vi "Create and Register Sessions.vi"(8 "error in (no error)":errorcluster, 11 "Pinmap Path":string) -> (0 "error out":errorcluster)   [LabVIEW 2020, in "NIDCPowerSourceDCVoltage.lvlib"]
uses:
  NIDCPowerSourceDCVoltage.lvlib
  <vilib>/MeasurementLink/MeasurementLink Session Management Client/RPC Messages/ni_measurementlink_sessionmanagement_v1_ReserveSessionsRequest.ctl
  <vilib>/MeasurementLink/MeasurementLink Session Management Client/RPC Messages/ni_measurementlink_PinMapContext.ctl
  <vilib>/MeasurementLink/MeasurementLink Discovery Client/RPC Messages/ni_measurementlink_discovery_v1_ResolveServiceRequest.ctl
  <vilib>/MeasurementLink/MeasurementLink Session Management Client/MeasurementLink Session Management Client.lvlib
  <vilib>/MeasurementLink/MeasurementLink Discovery Client/MeasurementLink Discovery Client.lvlib
  <vilib>/MeasurementLink/MeasurementLink Measurement Server/MeasurementLink Measurement Server.lvlib
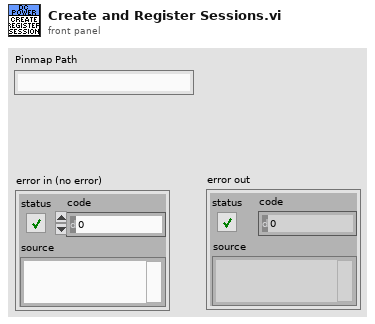
[diagram p1: front panel]
types:
  T1 = typedef "MeasurementLink Discovery Client.lvlib/ni_measurementlink_discovery_v1_ResolveServiceRequest.ctl" = cluster{"provided_interface":string, "service_class":string}
  T2 = typedef "MeasurementLink Session Management Client.lvlib/ni_measurementlink_sessionmanagement_v1_ReserveSessionsRequest.ctl" = cluster{"pin_map_context":T3, "pin_or_relay_names":string[], "instrument_type_id":string, "timeout_in_milliseconds":i32}
  T3 = typedef "MeasurementLink Session Management Client.lvlib/ni_measurementlink_PinMapContext.ctl" = cluster{"pin_map_id":string, "sites":i32[]}
  T4 = typedef "grpc-lvsupport-release.lvlib/grpcId.ctl" = u64
  T5 = typedef "MeasurementLink Discovery Client.lvlib/ni_measurementlink_discovery_v1_ServiceLocation.ctl" = cluster{"location":string, "insecure_port":string, "ssl_authenticated_port":string}
  T6 = typedef "MeasurementLink Session Management Client.lvlib/ni_measurementlink_sessionmanagement_v1_ReserveSessionsResponse.ctl" = cluster{"sessions":T7[]}
  T7 = typedef "MeasurementLink Session Management Client.lvlib/ni_measurementlink_sessionmanagement_v1_SessionInformation.ctl" = cluster{"session":T8, "resource_name":string, "channel_list":string, "instrument_type_id":string, "session_exists":bool, "channel_mappings":T9[]}
  T8 = typedef "MeasurementLink Session Management Client.lvlib/nidevice_grpc_Session.ctl" = cluster{"name":string}
  T9 = typedef "MeasurementLink Session Management Client.lvlib/ni_measurementlink_sessionmanagement_v1_ChannelMapping.ctl" = cluster{"pin_or_relay_name":string, "site":i32, "channel":string}
  T10 = typedef "niDCPower gRPC Device Server.ctl" = cluster{"session Name":string, "address (localhost)":string, "port (31763)":i32}
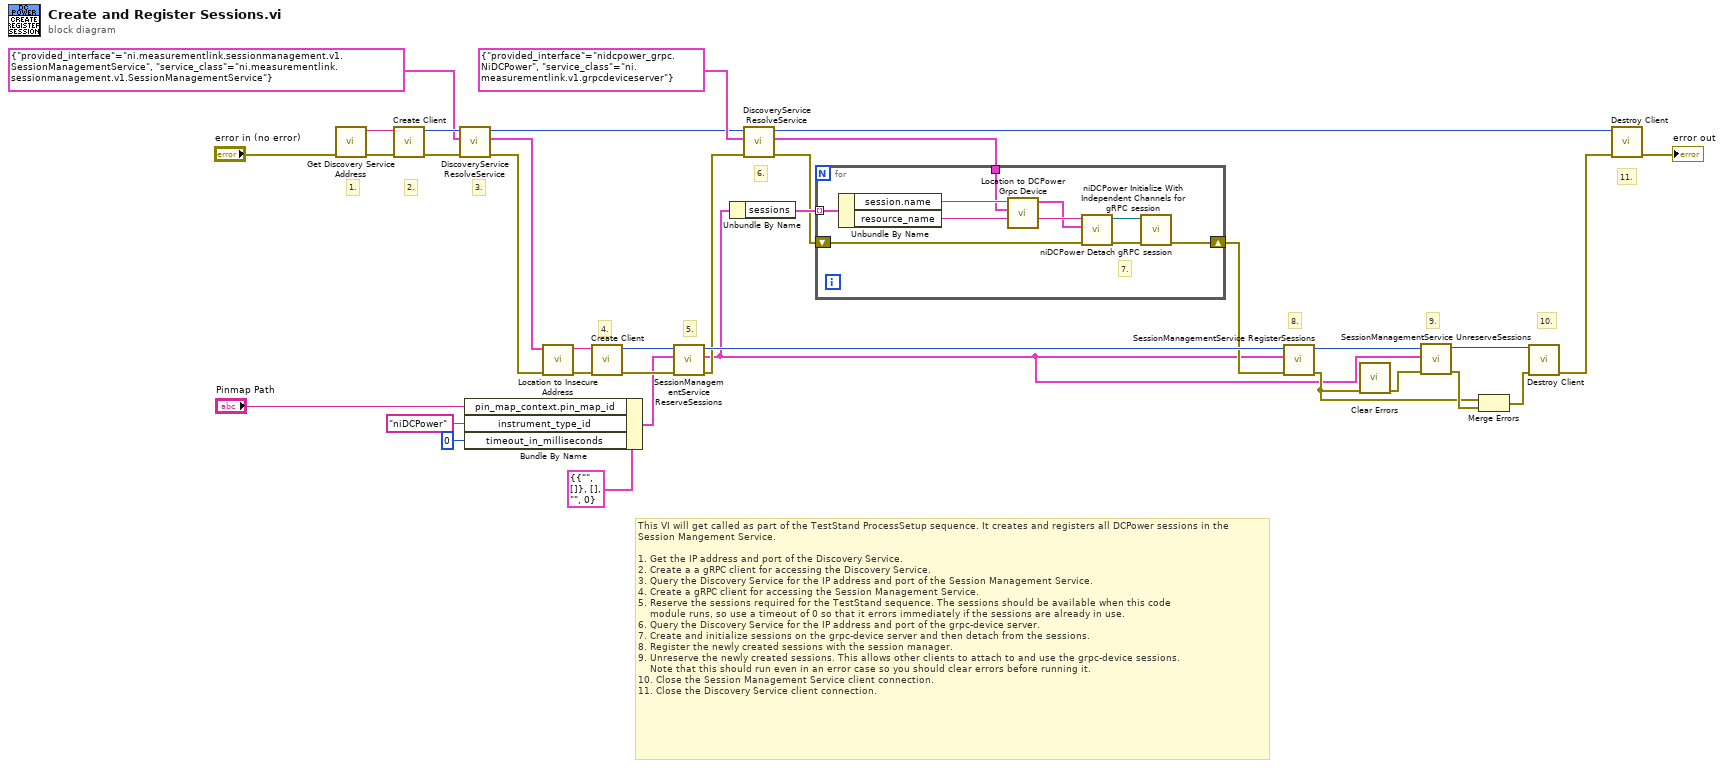
[diagram p0: block diagram]
diagram:
  # "11."
  # "10."
  # "9."
  # "8."
  # "6."
  # "5."
  # "4."
  # "3."
  # "2."
  # "1."
  # "This VI will get called as part of the TestStand ProcessSetup sequence. It creates and registers all DCPower sessions in the\nSession Mangement Service.\n\n1. Get the IP address and port of the Discovery Service.\n2. Create a a gRPC client for accessing the Discovery Service.\n3. Query the Discovery Service for the IP address and port of the Session Management Service.\n4. Create a gRPC client for accessing the Session Management Service.\n5. Reserve the sessions required for the TestStand sequence. The sessions should be available when this code\n    module runs, so use a timeout of 0 so that it errors immediately if the sessions are already in use.  \n6. Query the Discovery Service for the IP address and port of the grpc-device server.\n7. Create and initialize sessions on the grpc-device server and then detach from the sessions.\n8. Register the newly created sessions with the session manager.\n9. Unreserve the newly created sessions. This allows other clients to attach to and use the grpc-device sessions. \n    Note that this should run even in an error case so you should clear errors before running it.\n10. Close the Session Management Service client connection.\n11. Close the Discovery Service client connection."
  n1 = call <vilib>:"Get Discovery Service Address.vi"("error in"="error in (no error)") -> ("error out"=w10:errorcluster, "address"=w9:string)  [unwired: 9 in]
  n2 = call <vilib>:"Create Client.vi"("error in"=w10, "address"=w9) -> ("error out"=w30:errorcluster, "gRPC ID Out"=w31:T4)  [unwired: 8 in]
  n3 = call <vilib>:"DiscoveryService ResolveService.vi"("error in"=w30, "Request Data"=T1 {"provided_interface"="ni.measurementlink.sessionmanagement.v1.SessionManagementService", "service_class"="ni.measurementlink.sessionmanagement.v1.SessionManagementService"}, "gRPC ID"=w31) -> ("error out"=w29:errorcluster, "Response Data"=w8:T5, "gRPC ID out"=w17:T4)  [unwired: 6 in]
  n4 = Bundle By Name(cluster=T2 {"pin_map_context"={"pin_map_id"="", "sites"=[]}, "pin_or_relay_names"=[], "instrument_type_id"="", "timeout_in_milliseconds"=0} ("Request Data"), "pin_map_context.pin_map_id"="Pinmap Path", "instrument_type_id"="niDCPower", "timeout_in_milliseconds"=0) -> (w24:T2)
  n5 = call "Location to Insecure Address.vi"("Response Data"=w8) -> ("String"=w7:string)  [unwired: 10 in]
  n6 = call <vilib>:"Create Client.vi"("error in"=w29, "address"=w7) -> ("error out"=w33:errorcluster, "gRPC ID Out"=w34:T4)  [unwired: 8 in]
  n7 = call <vilib>:"SessionManagementService ReserveSessions.vi"("error in"=w33, "Request Data"=w24, "gRPC ID"=w34) -> ("error out"=w15:errorcluster, "Response Data"=w2:T6, "gRPC ID out"=w32:T4)  [unwired: 6 in]
  n8 = Unbundle By Name(w2) -> ("sessions"=w19:T7[])
  n9 = call <vilib>:"DiscoveryService ResolveService.vi"("error in"=w15, "Request Data"=T1 {"provided_interface"="nidcpower_grpc.NiDCPower", "service_class"="ni.measurementlink.v1.grpcdeviceserver"}, "gRPC ID"=w17) -> ("error out"=w14:errorcluster, "Response Data"=w13:T5, "gRPC ID out"=w16:T4)  [unwired: 6 in]
  n10 = for {
    tunnel: w19 -> [w40] mode=indexing
    shift-right: [w42] -> w22
    shift-left: w14 -> [w43]
    tunnel: w13 -> [w38]
    # "7."
    n11 = Unbundle By Name(w40) -> ("session.name"=w39:string, "resource_name"=w41:string)
    n12 = call "Location to DCPower Grpc Device.vi"("Grpc Device Location"=w38, "Session Name"=w39) -> ("NI gRPC Device Server Out"=w35:T10)  [unwired: 9 in]
    n13 = call <instrlib>:"niDCPower Initialize With Independent Channels for gRPC session.vi"("error in (no error)"=w43, "NI gRPC Device Server"=w35, "resource name"=w41) -> ("error out"=w37:errorcluster, "instrument handle out"=w36:refnum<k15>)  [unwired: 7 in]
    n14 = call <instrlib>:"niDCPower Detach gRPC session.vi"("error in (no error)"=w37, "instrument handle"=w36) -> ("error out"=w42:errorcluster)  [unwired: 9 in]
  }
  n15 = call <vilib>:"SessionManagementService RegisterSessions.vi"("error in"=w22, "Request Data"=w2, "gRPC ID"=w32) -> ("error out"=w3:errorcluster, "gRPC ID out"=w21:T4)  [unwired: 6 in, 1 out]
  n16 = call <vilib>:"Clear Errors.vi"("error in (no error)"=w3) -> ("error out"=w6:errorcluster)  [unwired: 5 in, 1 out]
  n17 = call <vilib>:"SessionManagementService UnreserveSessions.vi"("error in"=w6, "Request Data"=w2, "gRPC ID"=w21) -> ("error out"=w5:errorcluster, "gRPC ID out"=w20:T4)  [unwired: 6 in, 1 out]
  n18 = Merge Errors(w3, w5) -> (w4:errorcluster)
  n19 = call <vilib>:"Destroy Client.vi"("error in"=w4, "gRPC ID"=w20) -> ("error out"=w28:errorcluster)  [unwired: 9 in]
  n20 = call <vilib>:"Destroy Client.vi"("error in"=w28, "gRPC ID"=w16) -> ("error out"=→"error out":errorcluster)  [unwired: 9 in]
